vi "UI_Hit_Test.vi"(0 "X":i32, 5 "Y":i32, 7 "Specs":T1(array[cluster]), 9 "Dim Groups":bool[](array[boolean]), 11 "error in":errorcluster) -> (4 "Index":i32=-1, 6 "Group":i32=-1, 8 "Value":i32=-1, 15 "error out":errorcluster)   [LabVIEW 2026]
doc: "(X,Y)가 들어 있는 버튼 찾기. 없으면 Index/Group/Value = -1. 글자(Group -1)와 비활성 그룹은 제외."
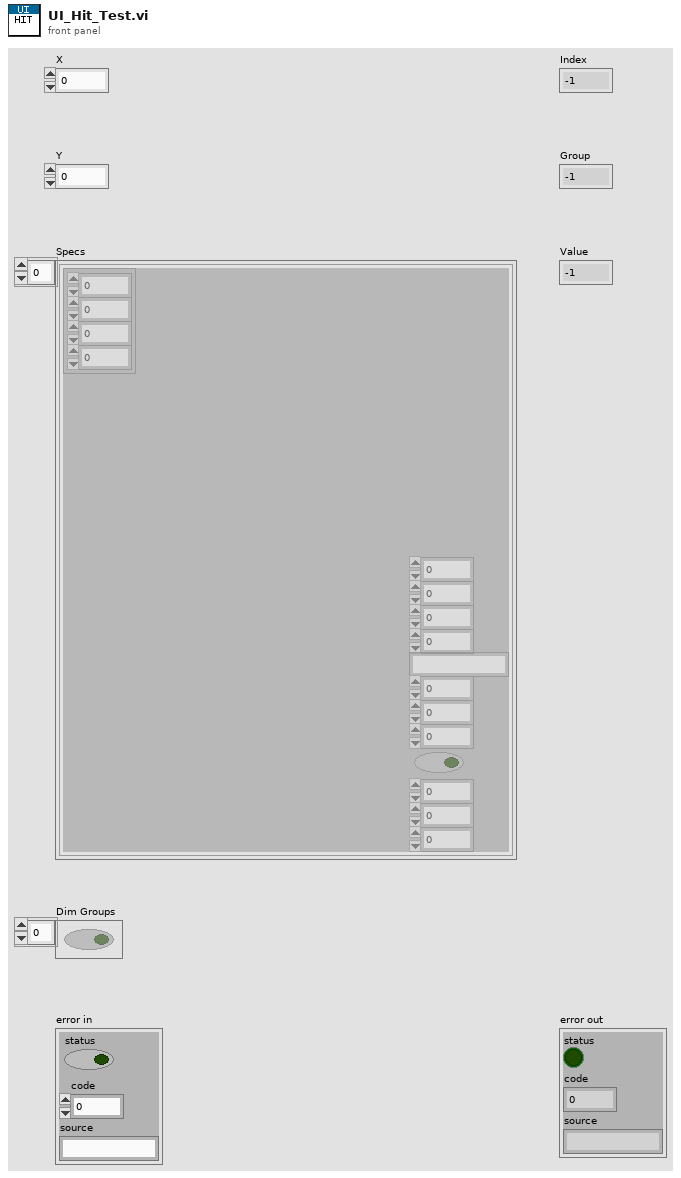
[diagram p1: front panel]
types:
  T1 = cluster{"Rect":cluster{"left":i16, "top":i16, "right":i16, "bottom":i16}, "Fill":u32, "Fill Sel":u32, "Border":u32, "Border Sel":u32, "Text":string, "Text Color":u32, "Text Sel":u32, "Size":i16, "Bold":bool, "Group":i32, "Value":i32, "Radius":i16}[]
  T2 = cluster{"left":i16, "top":i16, "right":i16, "bottom":i16}
  T3 = cluster{"Rect":cluster{"left":i16, "top":i16, "right":i16, "bottom":i16}, "Fill":u32, "Fill Sel":u32, "Border":u32, "Border Sel":u32, "Text":string, "Text Color":u32, "Text Sel":u32, "Size":i16, "Bold":bool, "Group":i32, "Value":i32, "Radius":i16}
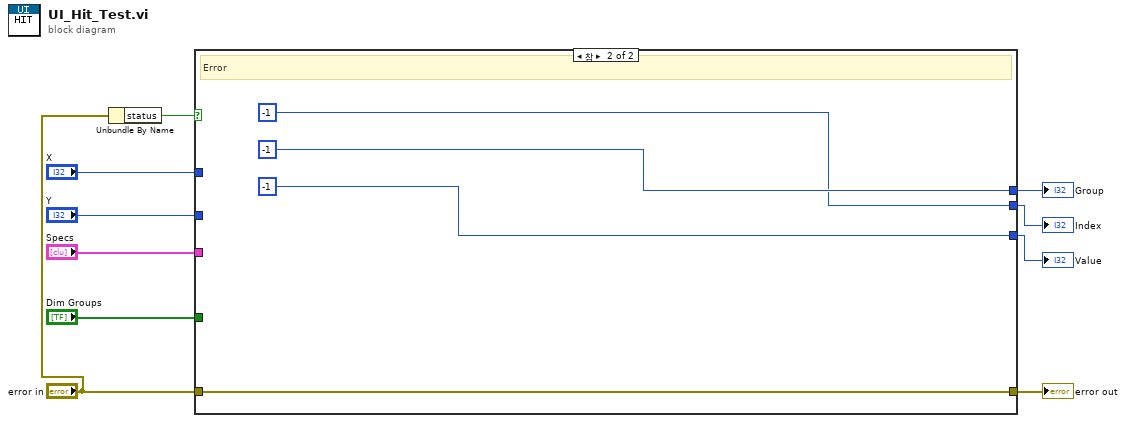
[diagram p0: block diagram]
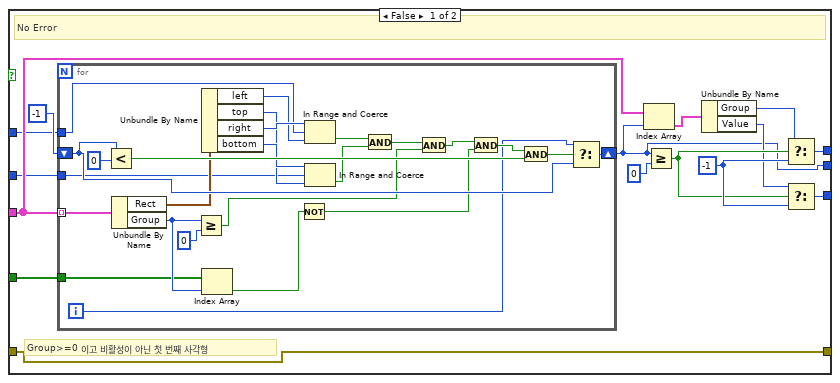
[diagram p2: hidden frame]
diagram:
  n1 = Unbundle By Name("error in") -> ("status"=w6:bool)
  n2 = case shown="참" w6 {
    tunnel: "X" -> [w11 _]
    tunnel: "Y" -> [w12 _]
    tunnel: "Specs" -> [w13 _]
    tunnel: "Dim Groups" -> [w14 _]
    tunnel: "error in" -> [w15 w51]
    tunnel: [w17 -1] -> w7
    tunnel: [w15 w51] -> w10
    tunnel: [w24 -1] -> w8
    tunnel: [w25 -1] -> w9
    frame False {
      w23 = -1
      # "Group>=0 이고 비활성이 아닌 첫 번째 사각형"
      # "No Error"
      n3 = for {
        shift-right: [w50] -> w17
        shift-left: -1 -> [w48]
        tunnel: w11 -> [w27]
        tunnel: w12 -> [w28]
        tunnel: w14 -> [w29]
        tunnel: w13 -> [w30] mode=indexing
        i -> [w26]
        n4 = Less?(x=w48, y=0) -> (x < y?=w47:bool)
        n5 = Unbundle By Name(w30) -> ("Rect"=w31:T2, "Group"=w32:i32)
        n6 = Greater Or Equal?(x=w32, y=0) -> (x >= y?=w41:bool)
        n7 = Unbundle By Name(w31) -> ("left"=w33:i16, "top"=w34:i16, "right"=w35:i16, "bottom"=w36:i16)
        n8 = Index Array(array=w29, index=w32) -> (element=w43:bool)
        n9 = Not(x=w43) -> (.not. x?=w44:bool)
        n10 = In Range and Coerce(upper limit=w35, x=w27, lower limit=w33) -> (In Range?=w37:bool)  [unwired: 1 out]
        n11 = In Range and Coerce(upper limit=w36, x=w28, lower limit=w34) -> (In Range?=w38:bool)  [unwired: 1 out]
        n12 = And(x=w37, y=w38) -> (x .and. y?=w39:bool)
        n13 = And(x=w39, y=w41) -> (x .and. y?=w42:bool)
        n14 = And(x=w42, y=w44) -> (x .and. y?=w45:bool)
        n15 = And(x=w45, y=w47) -> (x .and. y?=w49:bool)
        n16 = Select(t=w26, s=w49, f=w48) -> (s? t:f=w50:i32)
      }
      n17 = Index Array(array=w13, index=w17) -> (element=w18:T3)
      n18 = Greater Or Equal?(x=w17, y=0) -> (x >= y?=w22:bool)
      n19 = Unbundle By Name(w18) -> ("Group"=w19:i32, "Value"=w20:i32)
      n20 = Select(t=w19, s=w22, f=w23) -> (s? t:f=w24:i32)
      n21 = Select(t=w20, s=w22, f=w23) -> (s? t:f=w25:i32)
    }
    frame True {
      # "Error"
    }
  }
  "Index" <- w7
  "Group" <- w8
  "Value" <- w9
  "error out" <- w10
